vi "Prime Factors.vi"() -> ()   [LabVIEW 2026]
panel:
  out "Prime Factors":dbl[](array[numeric])
  in  "Input Number(N)":dbl
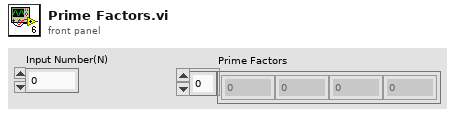
[diagram p1: front panel]
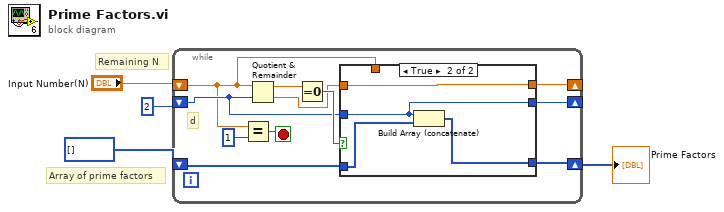
[diagram p0: block diagram]
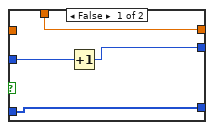
[diagram p2: hidden frame]
diagram:
  # "Array of prime factors"
  # "Remaining N"
  n1 = while {
    shift-right: [w10] -> _
    shift-left: "Input Number(N)" -> [w9]
    shift-right: [w12] -> _
    shift-left: 2 -> [w13]
    shift-right: [w5] -> w1
    shift-left: i32[] [] -> [w6]
    stop <- w7 stop-if-true
    # "d"
    n2 = Equal?(x=w9, y=1) -> (x = y?=w7:bool)
    n3 = Quotient & Remainder(x=w9, y=w13) -> (x-y*floor(x/y)=w15:dbl, floor(x/y)=w11:dbl)
    n4 = Equal To 0?(x=w15) -> (x = 0?=w14:bool)
    n5 = case shown="True" w14 {
      tunnel: w13 -> [w19 w21]
      tunnel: [w18 w21] -> w12
      tunnel: [w17 w23] -> w10
      tunnel: w11 -> [_ w23]
      tunnel: [w16 w22] -> w5
      tunnel: w9 -> [w17 _]
      tunnel: w6 -> [w16 w20]
      frame False {
        n6 = Increment(x=w19) -> (x+1=w18:i32)
      }
      frame True {
        n7 = Build Array (concatenate)(w21, w20) -> (w22:i32[])
      }
    }
  }
  "Prime Factors" <- w1
